vi "VibrationMonitoring.vi"() -> ()   [LabVIEW 2020]
uses:
  <vilib>/express/express analysis/Spectral/Block/exnSpectralBlock spectral measurements RMS poly.vi
  <vilib>/express/express analysis/Spectral/Block/exnSpectralBlock spectral measurements RMS DDT.vi
  <vilib>/express/express analysis/Spectral/XNode/ExpressSpectralMeasurementsBlockNode.xnode
panel:
  in  "stop":bool
  out "first subarray":bool[](array[boolean])
  out "FFT Graph":dynamicdata(graph)
  out "data":dynamicdata(graph)
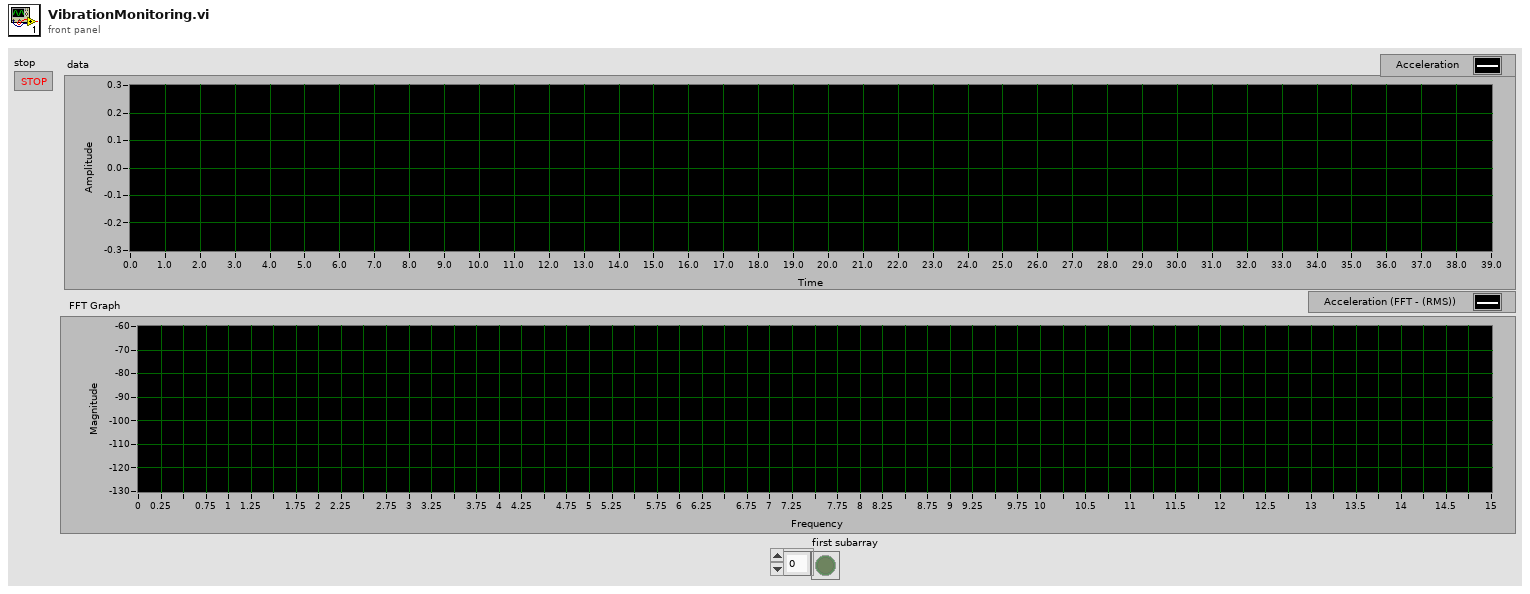
[diagram p1: front panel]
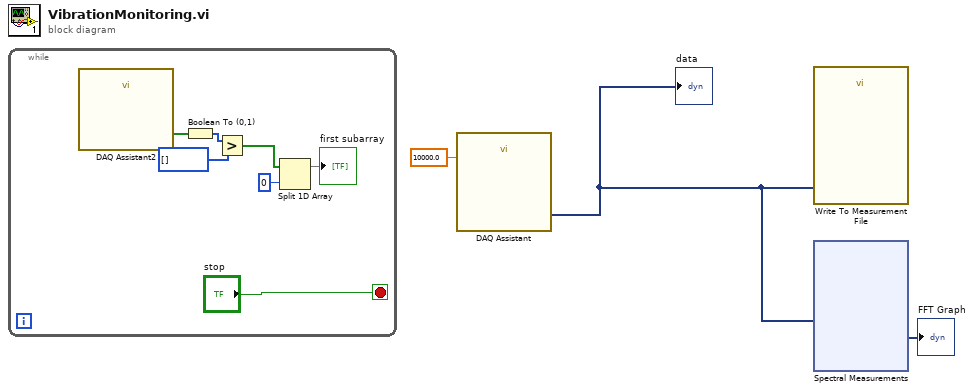
[diagram p0: block diagram]
diagram:
  n1 = while {
    stop <- "stop" stop-if-true
    n2 = call "DAQ Assistant2"() -> ("data"=w10:bool[])  [unwired: 17 in, 2 out]
    n3 = Boolean To (0,1)(Boolean=w10) -> (0, 1=w9:i16[])
    n4 = Greater?(x=w9, y=i16[] []) -> (0:w8:bool[])
    n5 = Split 1D Array(array=w8, index=0) -> (first subarray=→"first subarray":bool[])  [unwired: 1 out]
  }
  n6 = call "DAQ Assistant"("timeout (s)"=10000.0) -> ("data"=w3:dynamicdata)  [unwired: 16 in, 2 out]
  "data" <- w3
  n7 = call "Write To Measurement File"("Signals"=w3) -> ()  [unwired: 16 in, 3 out]
  n8 = xnode "Spectral Measurements"("Signals"=w3) -> ("FFT - (RMS)"=→"FFT Graph":dynamicdata)  [unwired: 1 in, 2 out]
